vi "Zero Phase Lowpass Filter (multiple).vi"(8 "error in (no error)":errorcluster, 10 "cutoff period (data)":dbl, 11 "XY-data":cluster{"X-array":dbl[], "Y-array":dbl[]}[](array[cluster])) -> (0 "error out":errorcluster, 3 "XY-data out":cluster{"X-array":dbl[], "Y-array":dbl[]}[](array[cluster]) {"Y-array" format="%.2p"; "X-array" format="%.2p"})   [LabVIEW 2019, in "xy_utilities.lvlib"]
doc: "Apply a Zero Phase Lowpass Filter to <b>XY-Data<b/>'s Y-Array.\n\n<b>cutoff period</b> is equivalent to 1/cutoff frequency and is in the units of the X-Array. The cutoff frequency is restricted between 0 and Fs/4.\n\nWire data to the data input to determine the polymorphic instance to use or manually select the instance."
uses:
  xy_utilities.lvlib
  Get X Array dx.vi
  <vilib>/Analysis/3filter.llb/FIR Windowed Coefficients.vi
  <vilib>/Analysis/3filter.llb/Zero Phase Filter.vi
  <vilib>/Analysis/3filter.llb/Zero Phase Filter (DBL).vi
  <vilib>/Utility/error.llb/Error Cluster From Error Code.vi
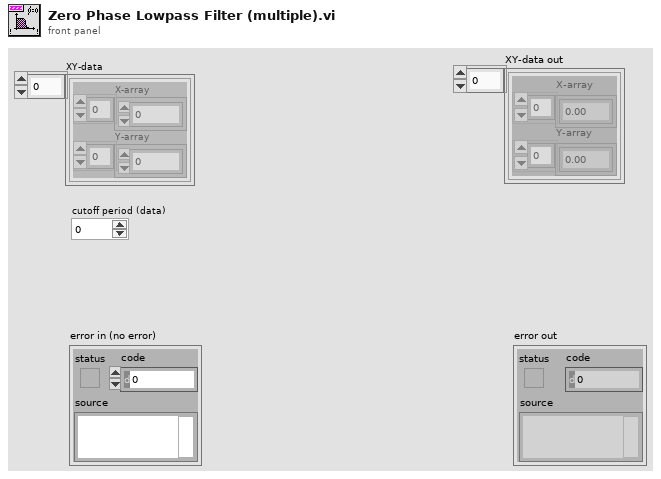
[diagram p1: front panel]
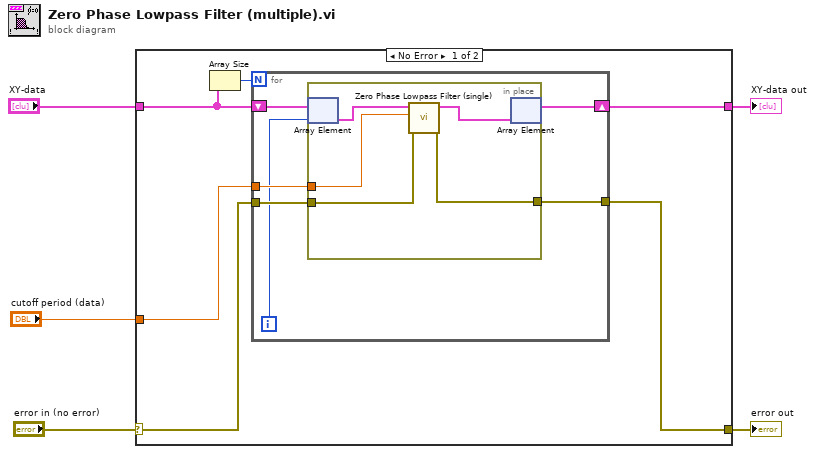
[diagram p0: block diagram]
diagram:
  n1 = case shown="No Error" "error in (no error)" {
    selector: "error in (no error)" -> [w9 w24]
    tunnel: [w8 w24] -> w4
    tunnel: "XY-data" -> [w6 w23]
    tunnel: [w11 w23] -> w2
    tunnel: "cutoff period (data)" -> [w10 _]
    frame No Error {
      n2 = Array Size(array=w6) -> (size(s)=w7:i32)
      n3 = for {
        N: w7 -> [_]
        tunnel: w10 -> [w17]
        tunnel: w9 -> [w16]
        tunnel: [w15] -> w8
        shift-right: [w12] -> w11
        shift-left: w6 -> [w13]
        i -> [w14]
        n4 = in-place {
          in-place-border: w17 -> [w22]
          in-place-border: w16 -> [w21]
          in-place-border: [w20] -> w15
          n5 = in-place-array #1(w13, w14) -> (w19:cluster{"X-array":dbl[], "Y-array":dbl[]})
          n6 = call "Zero Phase Lowpass Filter (single).vi"("error in (no error)"=w21, "cutoff period (data)"=w22, "XY-data"=w19) -> ("error out"=w20:errorcluster, "XY-data out"=w18:cluster{"X-array":dbl[], "Y-array":dbl[]})  [unwired: 7 in]
          n7 = in-place-array #1(w18) -> (w12:cluster{"X-array":dbl[], "Y-array":dbl[]}[])  [unwired: 1 out]
        }
      }
    }
    frame Error {
    }
  }
  "error out" <- w4
  "XY-data out" <- w2
